vi "Mink quadratic convert to J.vi"(10 "RawValCh1":dbl, 11 "Gentec Mlink.lvclass":refnum<class "Gentec Mlink.lvclass">) -> (2 "ScaledValueCh1":dbl, 3 "Gentec Mlink.lvclass":refnum<class "Gentec Mlink.lvclass">)   [LabVIEW 2020, in "Gentec Mlink.lvclass"]
uses:
  Gentec Mlink.lvclass
  Gentec Mlink.lvclass/Gentec Mlink.ctl
panel:
  out "error out":errorcluster
  in  "error in (no error)":errorcluster
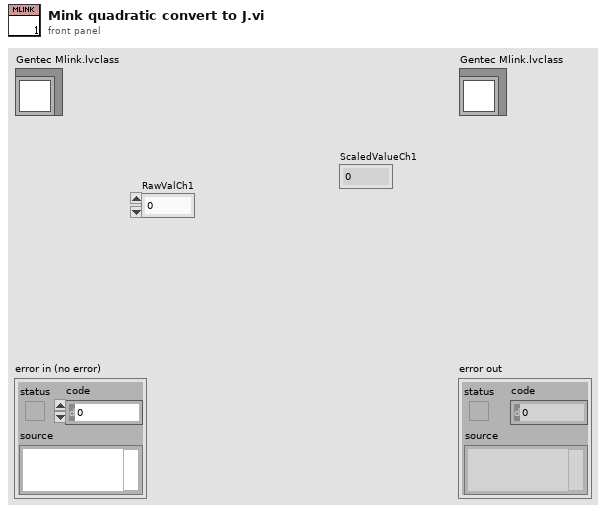
[diagram p1: front panel]
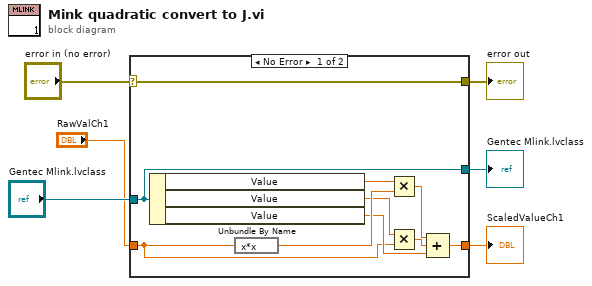
[diagram p0: block diagram]
diagram:
  n1 = case shown="No Error" "error in (no error)" {
    selector: "error in (no error)" -> [w16 w19]
    tunnel: [w16 w19] -> w5
    tunnel: [w9 w18] -> w3
    tunnel: "Gentec Mlink.lvclass" -> [w9 w18]
    tunnel: "RawValCh1" -> [w7 w17]
    tunnel: [w8 w17] -> w1
    frame No Error {
      n2 = Unbundle By Name(w9) -> ("Value"=w14:dbl, "Value"=w13:dbl, "Value"=w10:dbl)
      n3 = expression code="x*x"(w7) -> (w15:dbl)
      n4 = Multiply(x=w14, y=w15) -> (x*y=w12:dbl)
      n5 = Multiply(x=w13, y=w7) -> (x*y=w11:dbl)
      n6 = Compound Arithmetic op=ADD(w12, w11, w10) -> (w8:dbl)
    }
    frame Error {
    }
  }
  "error out" <- w5
  "Gentec Mlink.lvclass" <- w3
  "ScaledValueCh1" <- w1
